vi "Save to File.vi"(8 "error in":errorcluster, 10 "Folder":path, 11 "ILabVIEWFile in":refnum<class "Virtual Instrument.lvclass">) -> (0 "error out":errorcluster, 2 "File Path":path, 3 "ILabVIEWFile out":refnum<class "Virtual Instrument.lvclass">)   [LabVIEW 2026, in "Virtual Instrument.lvclass"]
doc: "Save VI in the provided folder. The file name is generated using the VIs name."
uses:
  Virtual Instrument.lvclass
  LabVIEW File/LabVIEW File.lvclass/LabVIEW File.ctl
  LabVIEW File/Read VI Reference.vi
  Virtual Instrument.lvclass/Virtual Instrument.ctl
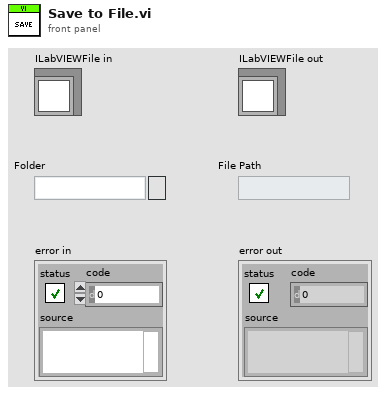
[diagram p1: front panel]
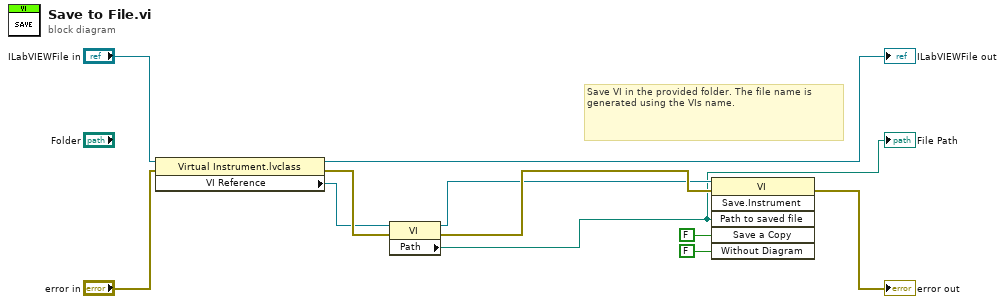
[diagram p0: block diagram]
diagram:
  # "Save VI in the provided folder. The file name is generated using the VIs name."
  n1 = property class="Virtual Instrument.lvclass"(reference="ILabVIEWFile in", error in="error in") -> (reference out=→"ILabVIEWFile out":refnum<class "Virtual Instrument.lvclass">, error out=w9:errorcluster, "VI Reference"=w3:refnum<vi>)
  n2 = property class="VI"(reference=w3, error in=w9) -> (reference out=w2:refnum<vi>, error out=w8:errorcluster, "Path"=w1:path)
  "File Path" <- w1
  n3 = invoke on="Invoke Node" class="VI" method="Save.Instrument"(reference=w2, error in=w8, "Path to saved file"=w1, "Save a Copy"=FALSE, "Without Diagram"=FALSE) -> (error out=→"error out":errorcluster)  [unwired: 1 in, 5 out]
